vi "Cmd_Dispatch.vi"(8 "error in":errorcluster, 10 "queue in":refnum<queue>, 11 "writer endpoint in":refnum<k21>) -> (0 "error Iout":errorcluster, 2 "queue out":refnum<queue>, 3 "writer endpoint out":refnum<k21>)   [LabVIEW 2025]
uses:
  vi/UI_Msg.ctl
  vi/action.ctl
  vi/thresholds.ctl
  vi/RT_Cmd.ctl
  vi/Command.ctl
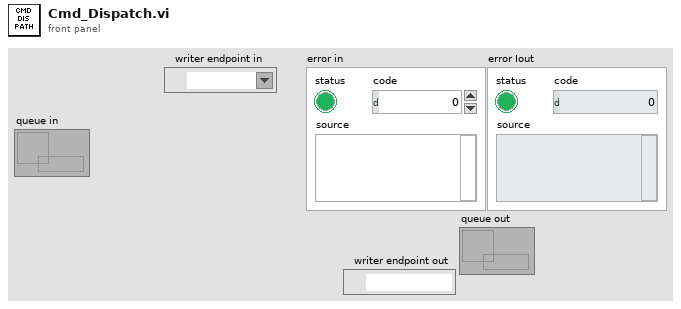
[diagram p1: front panel]
types:
  T1 = typedef "UI_Msg.ctl" = cluster{"action":T2, "Threshold":T3}
  T2 = typedef "action.ctl" = enum16{"Thresholds_Changed", "Manual_Trigger", "Stop"}
  T3 = typedef "thresholds.ctl" = cluster{"Thr_X":i16, "Thr_Y":i16, "Thr_Z":i16}
  T4 = typedef "Command.ctl" = enum16{"threshold_config", "manual_trigger", "stop", "remove_file"}
  T5 = typedef "RT_Cmd.ctl" = cluster{"command":T4, "parameters":T3}
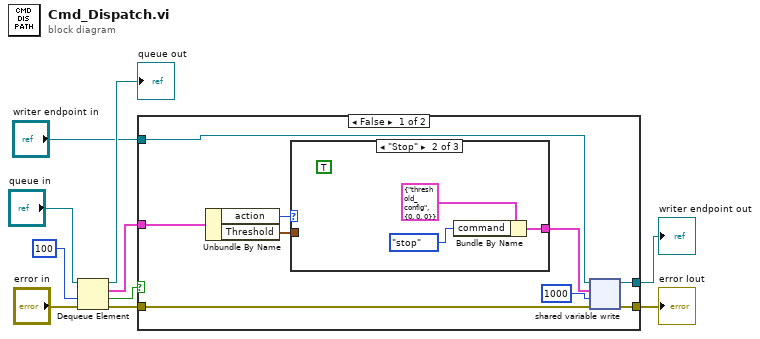
[diagram p0: block diagram]
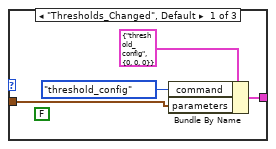
[diagram p2: hidden frame]
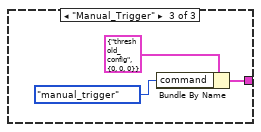
[diagram p3: hidden frame]
diagram:
  n1 = Dequeue Element(queue="queue in", timeout in ms (-1)=100, error in (no error)="error in") -> (queue out=→"queue out":refnum<queue>, element=w6:T1, timed out?=w7:bool, error out=w5:errorcluster)
  n2 = case shown="False" w7 {
    tunnel: w6 -> [w17 _]
    tunnel: w5 -> [w15 w30]
    tunnel: [w13 w30] -> w3
    tunnel: [w12 w31] -> w2
    tunnel: "writer endpoint in" -> [w11 w31]
    frame False {
      n3 = Unbundle By Name(w17) -> ("action"=w19:T2, "Threshold"=w18:T3)
      n4 = case shown="\"Stop\"" w19 {
        tunnel: [w21 w25 w28] -> w14
        tunnel: w18 -> [w22 _ _]
        frame "Thresholds_Changed", Default {
          (unwired) FALSE
          n5 = Bundle By Name(cluster=T5 {"command"=enum."threshold_config", "parameters"={"Thr_X"=0, "Thr_Y"=0, "Thr_Z"=0}} ("data"), "command"=Command."threshold_config", "parameters"=w22) -> (w21:T5)
        }
        frame "Stop" {
          (unwired) TRUE
          n6 = Bundle By Name(cluster=T5 {"command"=enum."threshold_config", "parameters"={"Thr_X"=0, "Thr_Y"=0, "Thr_Z"=0}} ("data"), "command"=Command."stop") -> (w25:T5)
        }
        frame "Manual_Trigger" {
          n7 = Bundle By Name(cluster=T5 {"command"=enum."threshold_config", "parameters"={"Thr_X"=0, "Thr_Y"=0, "Thr_Z"=0}} ("data"), "command"=Command."manual_trigger") -> (w28:T5)
        }
      }
      n8 = shared-variable-write(w11, w15, w14, 1000 ("timeout ms (-1)")) -> (w12:refnum<k21>, w13:errorcluster)  [unwired: 1 out]
    }
    frame True {
    }
  }
  "error Iout" <- w3
  "writer endpoint out" <- w2
